vi "Basic.vi"   [LabVIEW 2024]
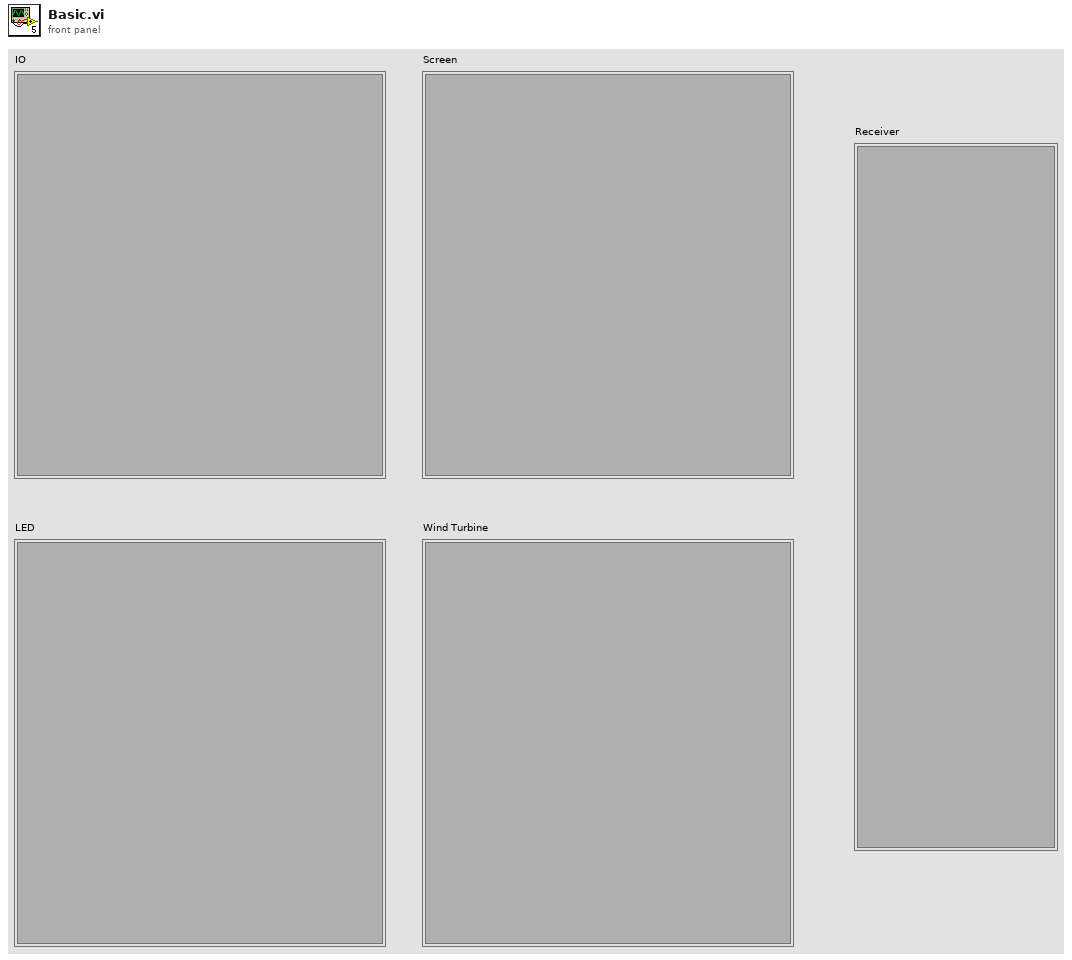
[diagram p1: front panel]
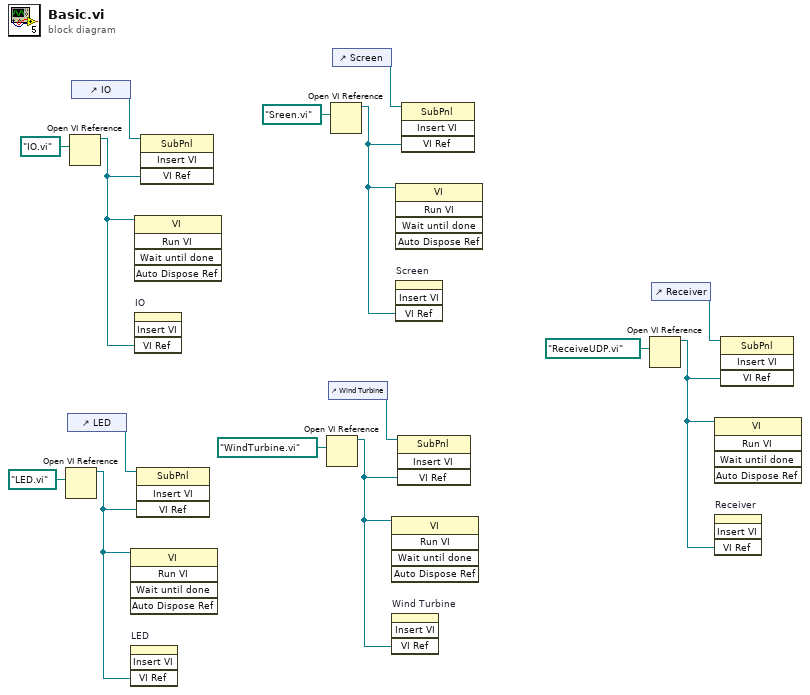
[diagram p0: block diagram]
diagram:
  n1 = Open VI Reference(vi path=path "LED.vi") -> (vi reference=w7:refnum<vi>)  [unwired: 5 in, 1 out]
  n2 = control-ref of="LED"() -> (w8:refnum<vi>)
  n3 = Open VI Reference(vi path=path "IO.vi") -> (vi reference=w13:refnum<vi>)  [unwired: 5 in, 1 out]
  n4 = control-ref of="IO"() -> (w14:refnum<vi>)
  n5 = invoke class="VI" method="Run VI"(reference=w7) -> ()  [unwired: 4 in, 5 out]
  n6 = invoke on="LED" class="SubPnl" method="Insert VI"("VI Ref"=w7) -> ()  [unwired: 3 in, 4 out]
  n7 = invoke class="VI" method="Run VI"(reference=w13) -> ()  [unwired: 4 in, 5 out]
  n8 = invoke on="IO" class="SubPnl" method="Insert VI"("VI Ref"=w13) -> ()  [unwired: 3 in, 4 out]
  n9 = invoke class="SubPnl" method="Insert VI"(reference=w8, "VI Ref"=w7) -> ()  [unwired: 2 in, 4 out]
  n10 = invoke class="SubPnl" method="Insert VI"(reference=w14, "VI Ref"=w13) -> ()  [unwired: 2 in, 4 out]
  n11 = Open VI Reference(vi path=path "WindTurbine.vi") -> (vi reference=w4:refnum<vi>)  [unwired: 5 in, 1 out]
  n12 = control-ref of="Wind Turbine"() -> (w5:refnum<vi>)
  n13 = Open VI Reference(vi path=path "Sreen.vi") -> (vi reference=w10:refnum<vi>)  [unwired: 5 in, 1 out]
  n14 = control-ref of="Screen"() -> (w11:refnum<vi>)
  n15 = invoke class="VI" method="Run VI"(reference=w4) -> ()  [unwired: 4 in, 5 out]
  n16 = invoke on="Wind Turbine" class="SubPnl" method="Insert VI"("VI Ref"=w4) -> ()  [unwired: 3 in, 4 out]
  n17 = invoke class="VI" method="Run VI"(reference=w10) -> ()  [unwired: 4 in, 5 out]
  n18 = invoke on="Screen" class="SubPnl" method="Insert VI"("VI Ref"=w10) -> ()  [unwired: 3 in, 4 out]
  n19 = invoke class="SubPnl" method="Insert VI"(reference=w5, "VI Ref"=w4) -> ()  [unwired: 2 in, 4 out]
  n20 = invoke class="SubPnl" method="Insert VI"(reference=w11, "VI Ref"=w10) -> ()  [unwired: 2 in, 4 out]
  n21 = Open VI Reference(vi path=path "ReceiveUDP.vi") -> (vi reference=w1:refnum<vi>)  [unwired: 5 in, 1 out]
  n22 = control-ref of="Receiver"() -> (w2:refnum<vi>)
  n23 = invoke class="VI" method="Run VI"(reference=w1) -> ()  [unwired: 4 in, 5 out]
  n24 = invoke on="Receiver" class="SubPnl" method="Insert VI"("VI Ref"=w1) -> ()  [unwired: 3 in, 4 out]
  n25 = invoke class="SubPnl" method="Insert VI"(reference=w2, "VI Ref"=w1) -> ()  [unwired: 2 in, 4 out]
